vi "ASD MIN over_S.vi"(8 "Right Read MIN":i32, 11 "AR BN#":i32[](array[numeric])) -> (3 "RR MIN Over S#":i32)   [LabVIEW 2018]
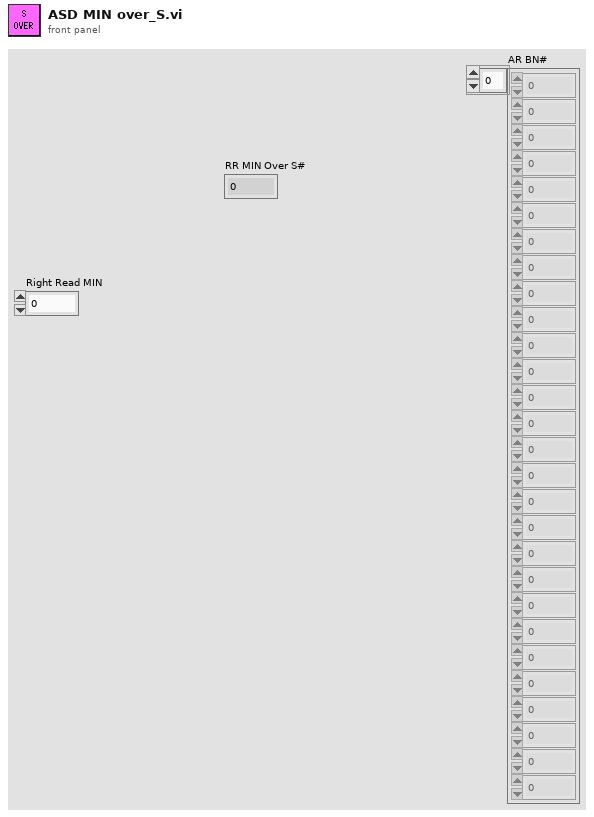
[diagram p1: front panel]
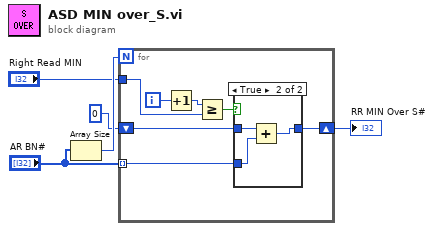
[diagram p0: block diagram]
diagram:
  n1 = Array Size(array="AR BN#") -> (size(s)=w5:i32)
  n2 = for {
    N: w5 -> [_]
    tunnel: "AR BN#" -> [w9] mode=indexing
    tunnel: "Right Read MIN" -> [w11]
    shift-right: [w8] -> w1
    shift-left: 0 -> [w7]
    i -> [w12]
    n3 = Increment(x=w12) -> (x+1=w6:i32)
    n4 = Greater Or Equal?(x=w6, y=w11) -> (x >= y?=w10:bool)
    n5 = case shown="True" w10 {
      tunnel: w9 -> [_ w14]
      tunnel: [w13 w16] -> w8
      tunnel: w7 -> [w13 w15]
      frame False {
      }
      frame True {
        n6 = Add(x=w15, y=w14) -> (x+y=w16:i32)
      }
    }
  }
  "RR MIN Over S#" <- w1
